vi "sub_panel_selection.vi"(8 "error in (no error) 2":errorcluster, 11 "reference":refnum<vi>) -> (0 "error out 2":errorcluster, 2 "Result":bool=TRUE)   [LabVIEW 2021]
uses:
  Control/Set_Get.ctl
panel:
  out "error out":errorcluster
  out "reference out":refnum<vi>
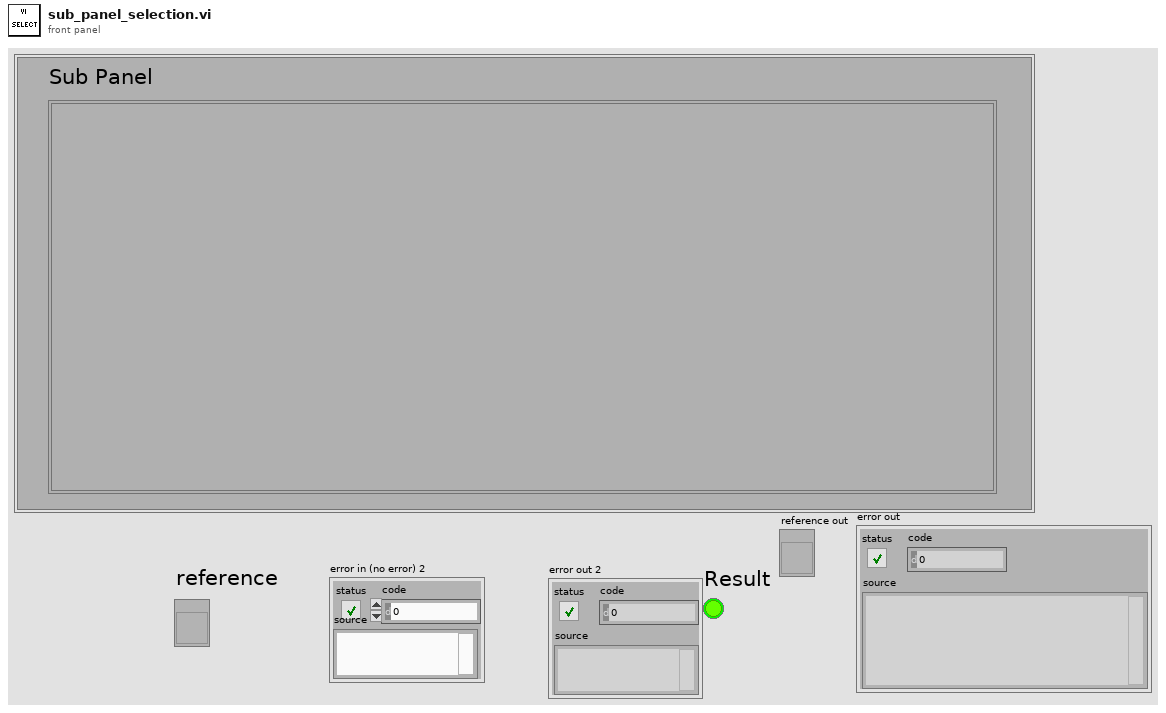
[diagram p1: front panel]
types:
  T1 = typedef "Set_Get.ctl" = enum16{"Set", "Get"}
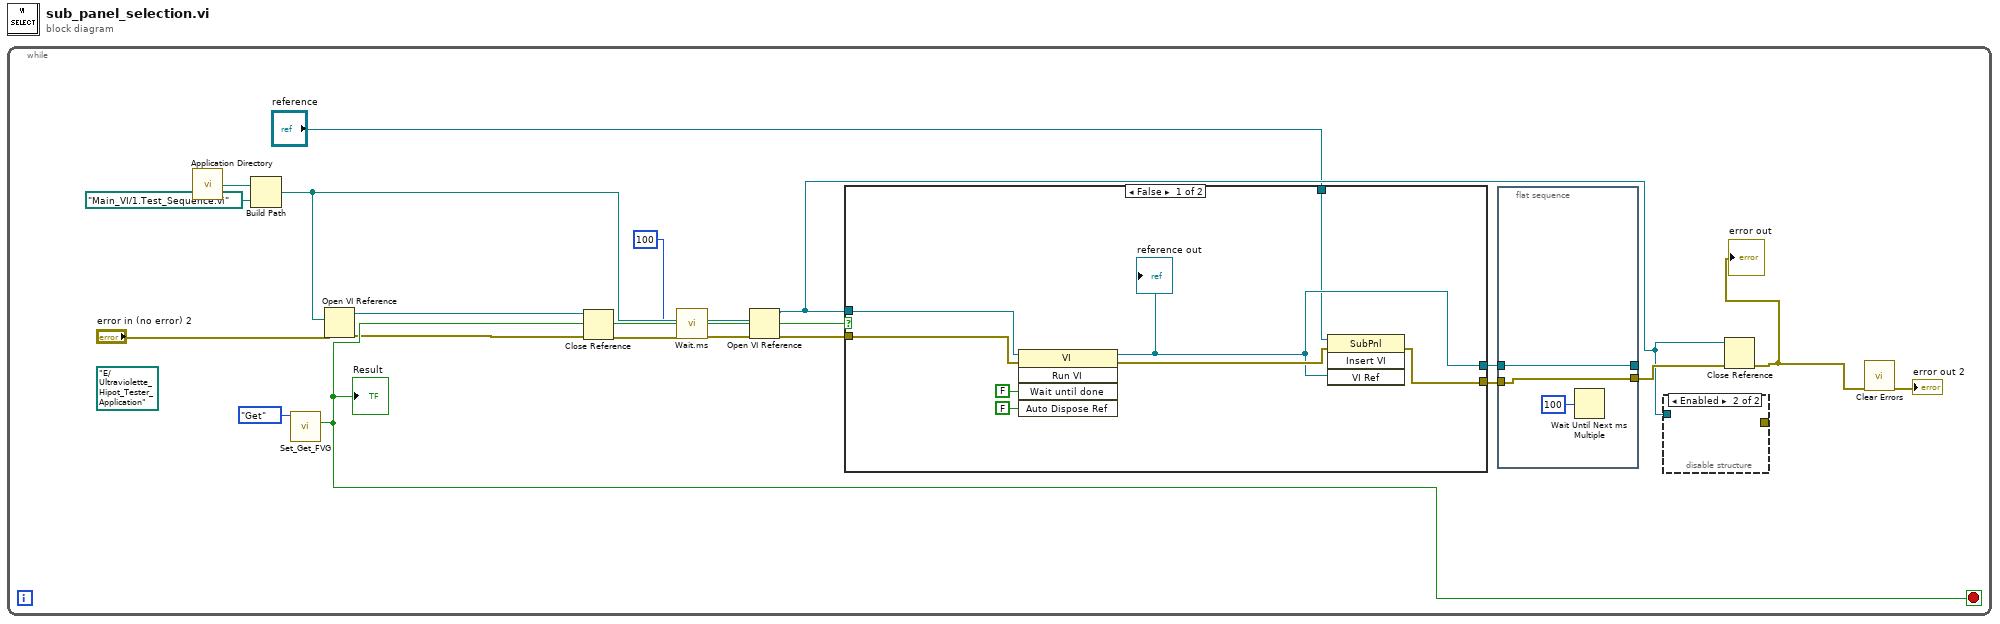
[diagram p0: block diagram]
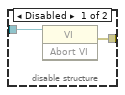
[diagram p2: hidden frame]
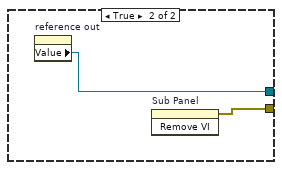
[diagram p3: hidden frame]
diagram:
  n1 = while {
    stop <- w10 stop-if-true
    (unwired) path "E:/Ultraviolette_Hipot_Tester_Application" ("vi path")
    n2 = call <vilib>:"Application Directory.vi"() -> ("Application Directory"=w16:path)
    n3 = Build Path(base path=w16, name or relative path=path "Main_VI/1.Test_Sequence.vi") -> (appended path=w9:path)
    n4 = call "Set_Get_FVG.vi"("Enum"=Set_Get."Get") -> ("Stop"=w10:bool)  [unwired: 10 in]
    "Result" <- w10
    n5 = Open VI Reference(vi path=w9, error in (no error)="error in (no error) 2") -> (vi reference=w5:refnum<vi>, error out=w1:errorcluster)  [unwired: 4 in]
    n6 = Close Reference(reference=w5, error in (no error)=w1) -> (error out=w4:errorcluster)
    n7 = call "Wait.ms.vi"("error in"=w4, "milliseconds to wait"=u32 100) -> ("error out"=w3:errorcluster)  [unwired: 9 in]
    n8 = Open VI Reference(vi path=w9, error in (no error)=w3) -> (vi reference=w8:refnum<vi>, error out=w7:errorcluster)  [unwired: 4 in]
    n9 = case shown="False" w10 {
      tunnel: [w30 w33] -> w13
      tunnel: [w28 w34] -> w14
      tunnel: w8 -> [w27 _]
      tunnel: "reference" -> [w26 _]
      tunnel: w7 -> [w25 _]
      frame False {
        n10 = invoke class="VI" method="Run VI"(reference=w27, error in=w25, "Wait until done"=FALSE ("Wait Until Done"), "Auto Dispose Ref"=FALSE ("Auto Dispose Reference")) -> (reference out=w28:refnum<vi>, error out=w29:errorcluster)  [unwired: 1 in, 3 out]
        "reference out" <- w28
        n11 = invoke on="Invoke Node" class="SubPnl" method="Insert VI"(reference=w26, error in=w29, "VI Ref"=w28) -> (error out=w30:errorcluster)  [unwired: 1 in, 3 out]
      }
      frame True {
        n12 = property on="reference out" class="VIRef (strict)"() -> ("Value"=w34:refnum<vi>)  [unwired: 2 in, 2 out]
        n13 = invoke on="Sub Panel" class="SubPnl" method="Remove VI"() -> (error out=w33:errorcluster)  [unwired: 3 in, 2 out]
      }
    }
    n14 = flat-sequence {
      tunnel: w14 -> [w21]
      tunnel: [w21] -> _
      tunnel: w13 -> [w20]
      tunnel: [w20] -> w12
      frame #0 {
        n15 = Wait Until Next ms Multiple(millisecond multiple=u32 100) -> ()  [unwired: 1 out]
      }
    }
    n16 = disable-structure shown="Enabled" {
      disable-tunnel: w8 -> [w24 _]
      disable-tunnel: [w23 _] -> _
      frame Disabled {
        n17 = invoke class="VI" method="Abort VI"(reference=w24) -> (error out=w23:errorcluster)  [unwired: 2 in, 2 out]
      }
      frame Enabled {
      }
    }
    n18 = Close Reference(reference=w8, error in (no error)=w12) -> (error out=w11:errorcluster)
    "error out" <- w11
    n19 = call <vilib>:"Clear Errors.vi"("error in (no error)"=w11) -> ("error out"=→"error out 2":errorcluster)  [unwired: 5 in, 1 out]
  }
